vi "Copy Template Files.vi"(8 "error in (no error)":errorcluster, 10 "Server Library (Library Item) in":refnum<vi>, 11 "Template Library (Library Item) in":refnum<vi>) -> (0 "error out":errorcluster, 2 "Server Library (Library Item) out":refnum<vi>, 3 "Template Library (Library Item) out":refnum<vi>)   [LabVIEW 2019, in "gRPC Template Creation Utility.lvlib"]
uses:
  gRPC Template Creation Utility.lvlib
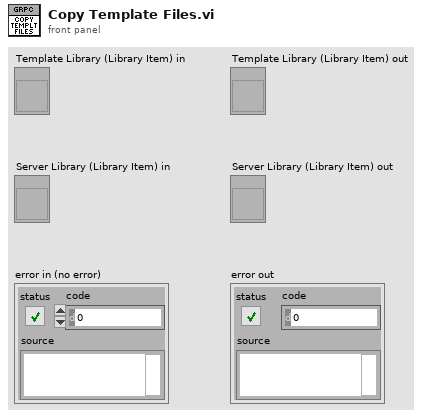
[diagram p1: front panel]
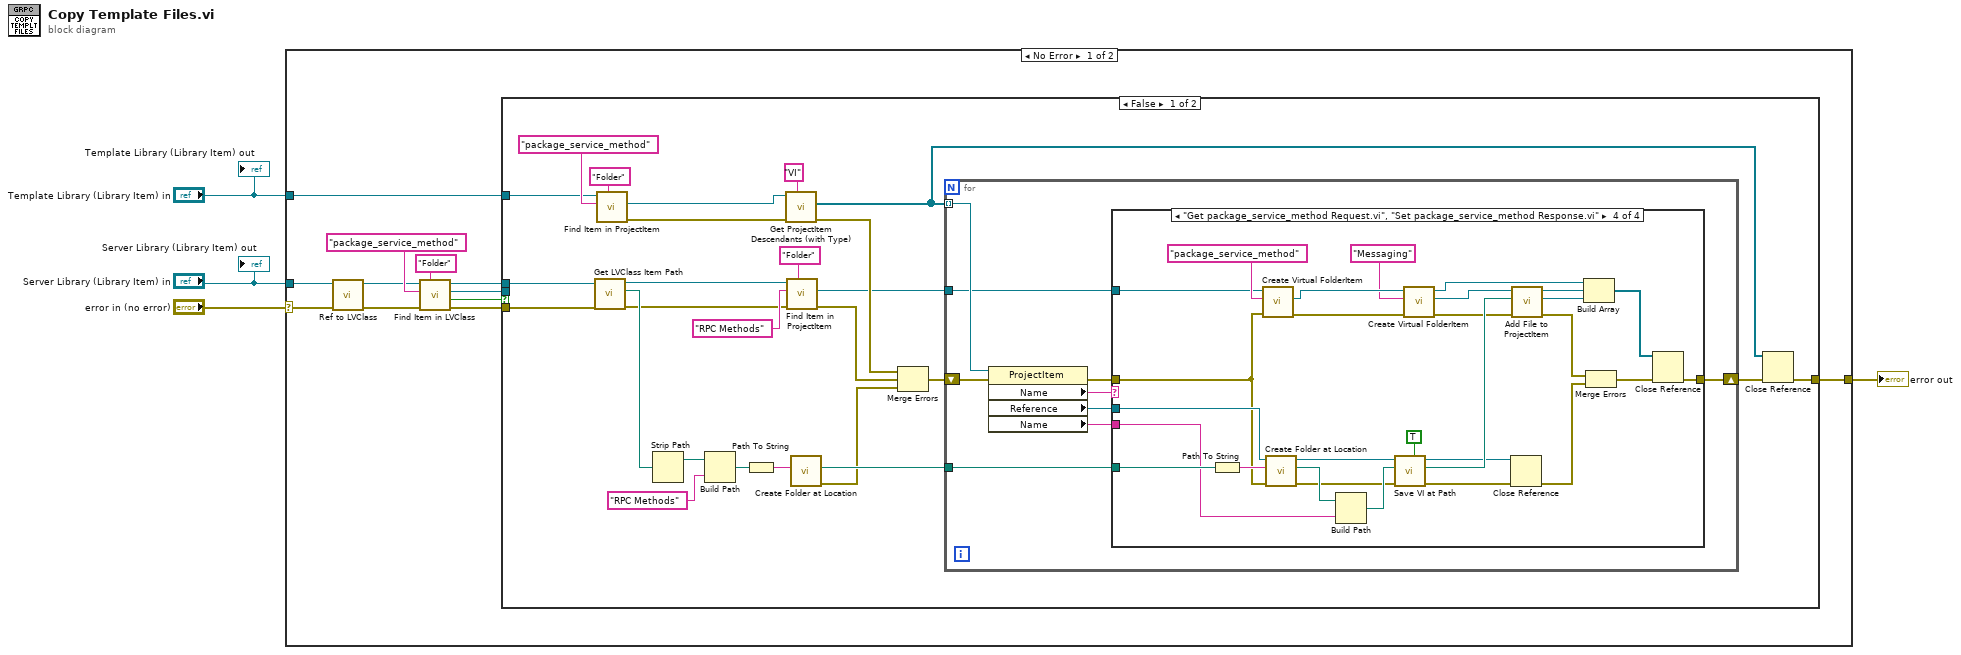
[diagram p0: block diagram]
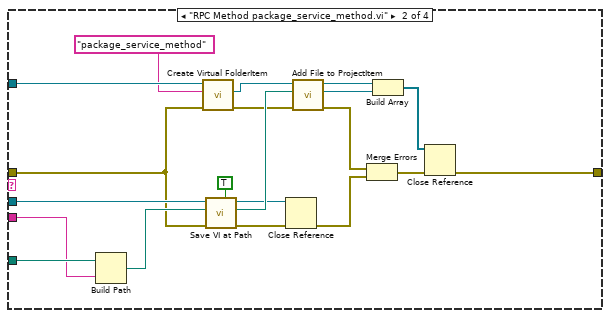
[diagram p3: hidden frame]
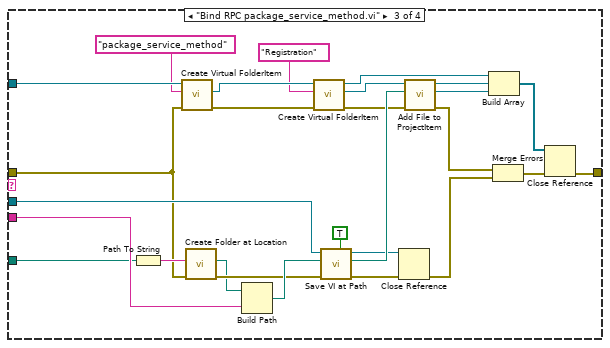
[diagram p4: hidden frame]
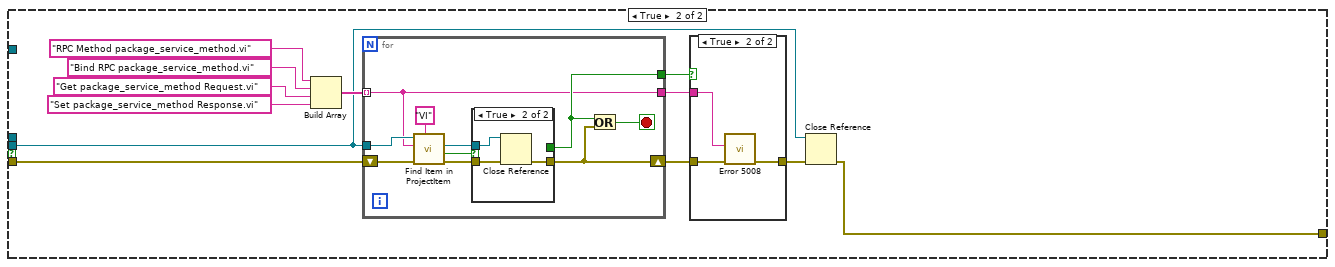
[diagram p5: hidden frame]
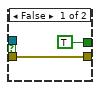
[diagram p7: hidden frame]
diagram:
  n1 = case shown="No Error" "error in (no error)" {
    selector: "error in (no error)" -> [w6 w158]
    tunnel: "Template Library (Library Item) in" -> [w9 _]
    tunnel: "Server Library (Library Item) in" -> [w8 _]
    tunnel: [w16 w158] -> w1
    frame No Error {
      n2 = call "Ref to LVClass.vi"("error in (no error)"=w6, "ProjectItem in"=w8) -> ("error out"=w5:errorcluster, "LVClassLibrary out"=w7:refnum<vi>)  [unwired: 8 in]
      n3 = call "Find Item in LVClass.vi"("Item Type"="Folder", "error in (no error)"=w5, "Item Name"="package_service_method" ("Name"), "Class Item in"=w7) -> ("error out"=w11:errorcluster, "Found?"=w13:bool, "Project Item (Class Item)"=w10:refnum<vi>, "Class Item out"=w12:refnum<vi>)  [unwired: 4 in]
      n4 = case shown="False" w13 {
        tunnel: w9 -> [w40 _]
        tunnel: [w23 w129] -> w16
        tunnel: w11 -> [w18 w127]
        tunnel: w12 -> [w19 _]
        tunnel: w10 -> [_ w128]
        frame False {
          n5 = call "Get LVClass Item Path.vi"("error in (no error)"=w18, "LVClassLibrary in"=w19) -> ("error out"=w20:errorcluster, "Path"=w22:path, "LVClassLibrary out"=w21:refnum<vi>)  [unwired: 7 in]
          n6 = call "Find Item in ProjectItem.vi"("Item Type"="Folder", "Name"="package_service_method", "ProjectItem in"=w40) -> ("error out"=w30:errorcluster, "Item Refnum out"=w39:refnum<vi>)  [unwired: 5 in, 2 out]
          n7 = Strip Path(path=w22) -> (stripped path=w37:path)  [unwired: 1 out]
          n8 = Build Path(base path=w37, name or relative path="RPC Methods") -> (appended path=w35:path)
          n9 = Path To String(path=w35) -> (string=w34:string)
          n10 = call "Get ProjectItem Descendants (with Type).vi"("Type"="VI", "error in (no error)"=w30, "ProjectItem in"=w39) -> ("error out"=w28:errorcluster, "All Descendents"=w17:refnum<vi>[])  [unwired: 6 in, 1 out]
          n11 = call "Find Item in ProjectItem.vi"("Item Type"="Folder", "error in (no error)"=w20, "Name"="RPC Methods", "ProjectItem in"=w21) -> ("error out"=w27:errorcluster, "Item Refnum out"=w25:refnum<vi>)  [unwired: 4 in, 2 out]
          n12 = call "Create Folder at Location.vi"("Path"=w34) -> ("Error Out"=w29:errorcluster, "Full path out"=w33:path)  [unwired: 8 in, 1 out]
          n13 = Merge Errors(w28, w27, w29) -> (w26:errorcluster)
          n14 = for {
            tunnel: w17 -> [w51] mode=indexing
            tunnel: w33 -> [w49]
            tunnel: w25 -> [w47]
            shift-right: [w43] -> w24
            shift-left: w26 -> [w45]
            n15 = property class="ProjectItem"(reference=w51, error in=w45) -> (error out=w44:errorcluster, "Name"=w50:string, "Reference"=w46:refnum<vi>, "Name"=w48:string)  [unwired: 1 out]
            n16 = case shown="\"Get package_service_method Request.vi\", \"Set package_service_method Response.vi\"" w50 {
              tunnel: w49 -> [_ w72 w97 w126]
              tunnel: w48 -> [_ w71 w99 w123]
              tunnel: w47 -> [_ w70 w91 w118]
              tunnel: w46 -> [_ w66 w96 w121]
              tunnel: w44 -> [w52 w63 w87 w114]
              tunnel: [w52 w56 w76 w104] -> w43
              frame "None", Default {
              }
              frame "RPC Method package_service_method.vi" {
                n17 = Build Path(base path=w72, name or relative path=w71) -> (appended path=w65:path)
                n18 = call "Create Virtual FolderItem.vi"("error in (no error)"=w63, "Folder Name"="package_service_method", "ProjectItem in"=w70) -> ("error out"=w62:errorcluster, "FolderItem reference out"=w68:refnum<vi>)  [unwired: 5 in, 2 out]
                n19 = call "Save VI at Path.vi"("Save a Copy (F)"=TRUE, "error in (no error)"=w63, "Path"=w65, "VI in"=w66) -> ("error out"=w55:errorcluster, "Path to saved File"=w64:path, "VI out"=w54:refnum<vi>)  [unwired: 5 in]
                n20 = Close Reference(reference=w54, error in (no error)=w55) -> (error out=w53:errorcluster)
                n21 = call "Add File to ProjectItem.vi"("error in (no error)"=w62, "File Path"=w64, "ProjectItem in"=w68) -> ("error out"=w61:errorcluster, "Added File ref"=w59:refnum<vi>, "ProjectItem out"=w60:refnum<vi>)  [unwired: 6 in]
                n22 = Merge Errors(w61, w53) -> (w58:errorcluster)
                n23 = Build Array(w60, w59) -> (w57:refnum<vi>[])
                n24 = Close Reference(reference=w57, error in (no error)=w58) -> (error out=w56:errorcluster)
              }
              frame "Bind RPC package_service_method.vi" {
                n25 = Path To String(path=w97) -> (string=w98:string)
                n26 = call "Create Virtual FolderItem.vi"("error in (no error)"=w87, "Folder Name"="package_service_method", "ProjectItem in"=w91) -> ("error out"=w86:errorcluster, "FolderItem reference out"=w93:refnum<vi>)  [unwired: 5 in, 2 out]
                n27 = call "Create Folder at Location.vi"("Error In"=w87, "Path"=w98) -> ("Error Out"=w84:errorcluster, "Full path out"=w83:path)  [unwired: 7 in, 1 out]
                n28 = Build Path(base path=w83, name or relative path=w99) -> (appended path=w94:path)
                n29 = call "Create Virtual FolderItem.vi"("error in (no error)"=w86, "Folder Name"="Registration", "ProjectItem in"=w93) -> ("error out"=w85:errorcluster, "FolderItem reference out"=w88:refnum<vi>, "ProjectItem out"=w80:refnum<vi>)  [unwired: 5 in, 1 out]
                n30 = call "Save VI at Path.vi"("Save a Copy (F)"=TRUE, "error in (no error)"=w84, "Path"=w94, "VI in"=w96) -> ("error out"=w75:errorcluster, "Path to saved File"=w89:path, "VI out"=w74:refnum<vi>)  [unwired: 5 in]
                n31 = Close Reference(reference=w74, error in (no error)=w75) -> (error out=w73:errorcluster)
                n32 = call "Add File to ProjectItem.vi"("error in (no error)"=w85, "File Path"=w89, "ProjectItem in"=w88) -> ("error out"=w82:errorcluster, "Added File ref"=w78:refnum<vi>, "ProjectItem out"=w79:refnum<vi>)  [unwired: 6 in]
                n33 = Build Array(w80, w79, w78) -> (w77:refnum<vi>[])
                n34 = Merge Errors(w82, w73) -> (w81:errorcluster)
                n35 = Close Reference(reference=w77, error in (no error)=w81) -> (error out=w76:errorcluster)
              }
              frame "Get package_service_method Request.vi", "Set package_service_method Response.vi" {
                n36 = Path To String(path=w126) -> (string=w125:string)
                n37 = call "Create Virtual FolderItem.vi"("error in (no error)"=w114, "Folder Name"="package_service_method", "ProjectItem in"=w118) -> ("error out"=w112:errorcluster, "FolderItem reference out"=w117:refnum<vi>)  [unwired: 5 in, 2 out]
                n38 = call "Create Folder at Location.vi"("Error In"=w114, "Path"=w125) -> ("Error Out"=w113:errorcluster, "Full path out"=w124:path)  [unwired: 7 in, 1 out]
                n39 = Build Path(base path=w124, name or relative path=w123) -> (appended path=w120:path)
                n40 = call "Save VI at Path.vi"("Save a Copy (F)"=TRUE, "error in (no error)"=w113, "Path"=w120, "VI in"=w121) -> ("error out"=w103:errorcluster, "Path to saved File"=w115:path, "VI out"=w102:refnum<vi>)  [unwired: 5 in]
                n41 = call "Create Virtual FolderItem.vi"("error in (no error)"=w112, "Folder Name"="Messaging", "ProjectItem in"=w117) -> ("error out"=w111:errorcluster, "FolderItem reference out"=w108:refnum<vi>, "ProjectItem out"=w109:refnum<vi>)  [unwired: 5 in, 1 out]
                n42 = Close Reference(reference=w102, error in (no error)=w103) -> (error out=w101:errorcluster)
                n43 = call "Add File to ProjectItem.vi"("error in (no error)"=w111, "File Path"=w115, "ProjectItem in"=w108) -> ("error out"=w110:errorcluster, "Added File ref"=w107:refnum<vi>, "ProjectItem out"=w100:refnum<vi>)  [unwired: 6 in]
                n44 = Build Array(w109, w100, w107) -> (w105:refnum<vi>[])
                n45 = Merge Errors(w110, w101) -> (w106:errorcluster)
                n46 = Close Reference(reference=w105, error in (no error)=w106) -> (error out=w104:errorcluster)
              }
            }
          }
          n47 = Close Reference(reference=w17, error in (no error)=w24) -> (error out=w23:errorcluster)
        }
        frame True {
          n48 = Build Array("RPC Method package_service_method.vi" ("Name"), "Bind RPC package_service_method.vi" ("element"), "Get package_service_method Request.vi" ("element"), "Set package_service_method Response.vi" ("element")) -> (w134:string[])
          n49 = for {
            tunnel: w128 -> [w152]
            tunnel: w134 -> [w143] mode=indexing
            shift-right: [w145] -> w133
            shift-left: w127 -> [w148]
            tunnel: [w144] -> w132
            tunnel: [w143] -> w131
            stop <- w146 stop-if-true
            n50 = call "Find Item in ProjectItem.vi"("Item Type"="VI", "error in (no error)"=w148, "Name"=w143, "ProjectItem in"=w152) -> ("error out"=w147:errorcluster, "Found ?"=w150:bool, "Item Refnum out"=w149:refnum<vi>)  [unwired: 4 in, 1 out]
            n51 = case shown="True" w150 {
              tunnel: w149 -> [_ w157]
              tunnel: w147 -> [w154 w156]
              tunnel: [w154 w155] -> w145
              tunnel: [TRUE _] -> w144
              frame False {
              }
              frame True {
                n52 = Close Reference(reference=w157, error in (no error)=w156) -> (error out=w155:errorcluster)
              }
            }
            n53 = Or(x=w144, y=w145) -> (x .or. y?=w146:bool)
          }
          n54 = case shown="True" w132 {
            tunnel: w133 -> [w139 w142]
            tunnel: w131 -> [_ w141]
            tunnel: [w139 w140] -> w130
            frame False {
            }
            frame True {
              n55 = call "Error 5008.vi"("error in (no error)"=w142, "File Name"=w141) -> ("error out"=w140:errorcluster)  [unwired: 9 in]
            }
          }
          n56 = Close Reference(reference=w128, error in (no error)=w130) -> (error out=w129:errorcluster)
        }
      }
    }
    frame Error {
    }
  }
  "error out" <- w1
  "Template Library (Library Item) out" <- "Template Library (Library Item) in"
  "Server Library (Library Item) out" <- "Server Library (Library Item) in"
